vi "Check Events.vi"(8 "error in (no error)":errorcluster, 11 "PluginGUI in":refnum<class "PluginGUI.lvclass">) -> (0 "error out":errorcluster, 3 "PluginGUI out":refnum<class "PluginGUI.lvclass">)   [LabVIEW 2020, in "VolatusGUI.lvlib" / "PluginGUI.lvclass"]
uses:
  PluginGUI.lvclass
  C:/dev/lv20CE/relink/lv-volatus/Volatus/Module/Module.lvclass
  PluginGUI.lvclass/PluginGUI.ctl
  Volatus/Module/Module.lvclass/Module.ctl
  OnValueChangeHandler/OnValueChangeHandler.lvclass
  OnMouseDown/OnMouseDown.lvclass
  Volatus/Module/Module.lvclass
  Volatus/VolatusAPI/VolatusAPI.lvclass
  Volatus/Volatus.lvlib
  C:/dev/lv20CE/relink/lv-volatus/VolatusGUI/PluginGUI/PluginGUI.lvclass
  GUI Helper/GUI Helper.lvclass
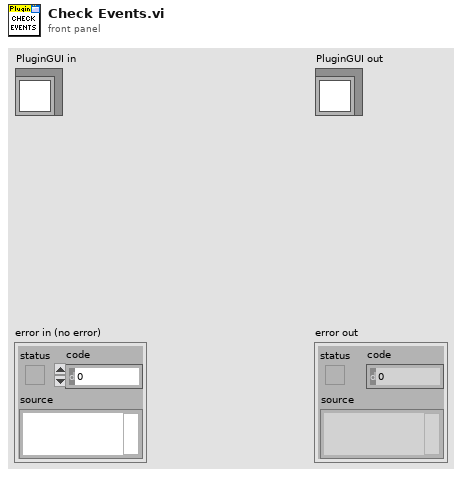
[diagram p1: front panel]
types:
  T1 = typedef "LVPoint32TypeDef.ctl" = cluster{"Horizontal":i32, "Vertical":i32}
  T2 = cluster{"Shift":bool, "Ctrl":bool, "Alt":bool, "Cmd":bool, "Opt":bool}
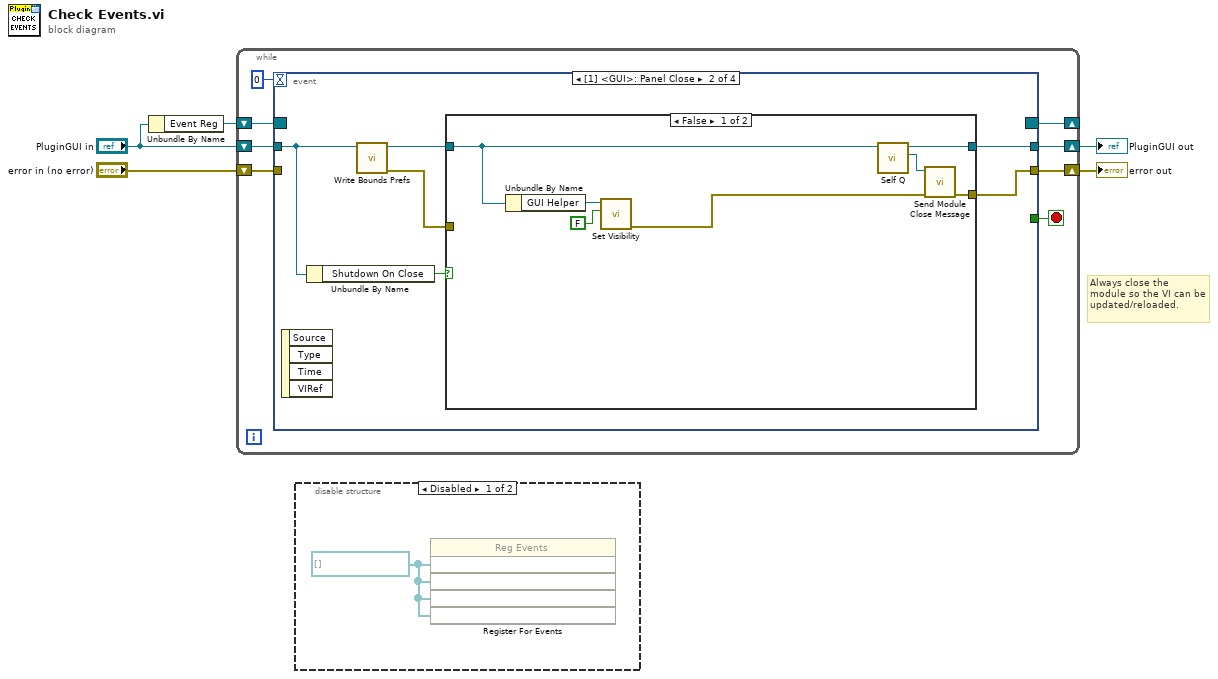
[diagram p0: block diagram]
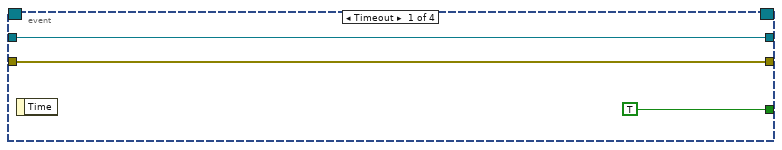
[diagram p3: hidden frame]
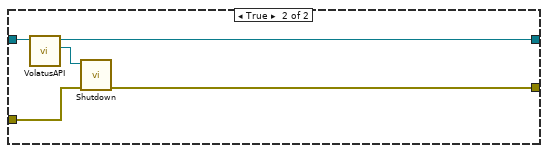
[diagram p4: hidden frame]
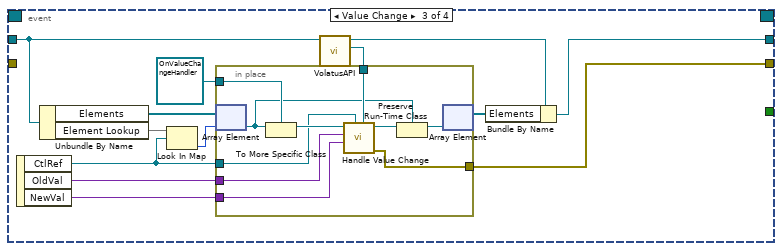
[diagram p5: hidden frame]
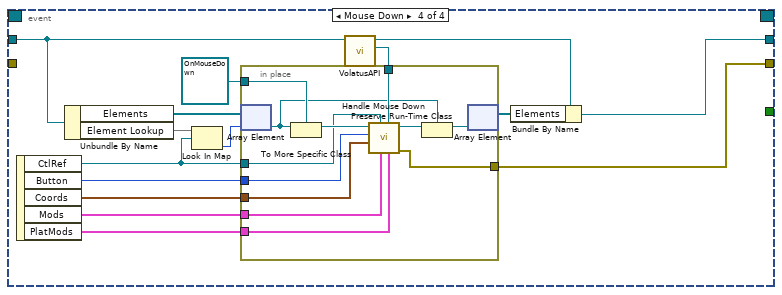
[diagram p6: hidden frame]
diagram:
  # "Always close the module so the VI can be updated/reloaded."
  n1 = Unbundle By Name("PluginGUI in") -> ("Event Reg"=w4:refnum<event-registration>)
  n2 = while {
    shift-right: [w8] -> w2
    shift-left: "PluginGUI in" -> [w11]
    shift-right: [w12] -> _
    shift-left: w4 -> [w13]
    shift-right: [w7] -> w1
    shift-left: "error in (no error)" -> [w10]
    stop <- w6 stop-if-true
    n3 = event shown="[1] <GUI>: Panel Close" {
      selector: w13 -> [_ _ _ _]
      dyn-events: [_ _ _ _] -> w12
      timeout: 0 -> [_ _ _ _]
      tunnel: w11 -> [w16 w21 w42 w58]
      tunnel: w10 -> [w15 _ _ _]
      tunnel: [w16 w20 w36 w64] -> w8
      tunnel: [w15 w19 w37 w65] -> w7
      tunnel: [TRUE _ _ _] -> w6
      event Timeout {
        n4 = event-data() -> ()  [unwired: 1 in, 1 out]
      }
      event Panel Close {
        n5 = event-data() -> ()  [unwired: 1 in, 4 out]
        n6 = Unbundle By Name(w21) -> ("Shutdown On Close"=w22:bool)
        n7 = call "Write Bounds Prefs.vi"("PluginGUI in"=w21) -> ("error out"=w17:errorcluster, "PluginGUI out"=w18:refnum<class "PluginGUI.lvclass">)  [unwired: 9 in]
        n8 = case shown="False" w22 {
          tunnel: w18 -> [w26 w34]
          tunnel: [w29 w32] -> w20
          tunnel: [w27 w31] -> w19
          tunnel: w17 -> [_ w30]
          frame False {
            n9 = Unbundle By Name(w26) -> ("GUI Helper"=w25:refnum<class "MessageQ.lvclass">)
            n10 = call "Set Visibility.vi"("Visible"=FALSE, "GUI Helper in"=w25) -> ("error out"=w23:errorcluster)  [unwired: 8 in, 1 out]
            n11 = call "Self Q.vi"("Module in"=w26) -> ("Self Q"=w28:refnum<class "MessageQ.lvclass">, "Module in"=w29:refnum<class "PluginGUI.lvclass">)  [unwired: 9 in]
            n12 = call "Send Module Close Message.vi"("error in (no error)"=w23, "MessageQ"=w28) -> ("error out"=w27:errorcluster)  [unwired: 9 in]
          }
          frame True {
            n13 = call "VolatusAPI.vi"("Module in"=w34) -> ("VolatusAPI"=w33:refnum<class "VolatusAPI.lvclass">, "Module in"=w32:refnum<class "PluginGUI.lvclass">)  [unwired: 9 in]
            n14 = call "Shutdown.vi"("error in (no error)"=w30, "VolatusAPI in"=w33) -> ("error out"=w31:errorcluster)  [unwired: 8 in, 1 out]
          }
        }
      }
      event Value Change {
        n15 = event-data() -> ("CtlRef"=w43:refnum<vi>, "OldVal"=w39:variant, "NewVal"=w38:variant)  [unwired: 1 in]
        n16 = Unbundle By Name(w42) -> ("Elements"=w46:refnum<class "GUI Element.lvclass">[], "Element Lookup"=w47:map{refnum<vi>, i32})
        n17 = Look In Map(map=w47, key=w43) -> (value=w45:i32)  [unwired: 1 in, 1 out]
        n18 = call "VolatusAPI.vi"("Module in"=w42) -> ("VolatusAPI"=w41:refnum<class "VolatusAPI.lvclass">, "Module in"=w40:refnum<class "PluginGUI.lvclass">)  [unwired: 9 in]
        n19 = in-place {
          in-place-border: refnum<class "OnValueChangeHandler.lvclass"> refnum ("OnValueChangeHandler in") -> [w56]
          in-place-border: w43 -> [w55]
          in-place-border: w41 -> [w54]
          in-place-border: w39 -> [w53]
          in-place-border: w38 -> [w52]
          in-place-border: [w48] -> w37
          n20 = in-place-array #1(w46, w45) -> (w49:refnum<class "GUI Element.lvclass">)
          n21 = To More Specific Class(target class=w56, reference=w49) -> (specific class reference=w57:refnum<class "OnValueChangeHandler.lvclass">)  [unwired: 1 in, 1 out]
          n22 = call-dynamic "Handle Value Change.vi"("VolatusAPI"=w54, "CtlRef"=w55, "NewVal"=w52, "OldVal"=w53, "OnValueChangeHandler in"=w57) -> ("error out"=w48:errorcluster, "OnValueChangeHandler out"=w51:refnum<class "OnValueChangeHandler.lvclass">)  [unwired: 5 in]
          n23 = Preserve Run-Time Class(object in=w51, 2:w49) -> (object out=w50:refnum<class "GUI Element.lvclass">)  [unwired: 1 in, 1 out]
          n24 = in-place-array #1(w50) -> (w35:refnum<class "GUI Element.lvclass">[])  [unwired: 1 out]
        }
        n25 = Bundle By Name(cluster=w40, "Elements"=w35) -> (w36:refnum<class "PluginGUI.lvclass">)
      }
      event Mouse Down {
        n26 = event-data() -> ("CtlRef"=w63:refnum<vi>, "Button"=w62:u16, "Coords"=w61:T1, "Mods"=w60:cluster{"Double Click":bool, "Menu Key":bool}, "PlatMods"=w59:T2)  [unwired: 1 in]
        n27 = Unbundle By Name(w58) -> ("Elements"=w71:refnum<class "GUI Element.lvclass">[], "Element Lookup"=w72:map{refnum<vi>, i32})
        n28 = Look In Map(map=w72, key=w63) -> (value=w70:i32)  [unwired: 1 in, 1 out]
        n29 = call "VolatusAPI.vi"("Module in"=w58) -> ("VolatusAPI"=w68:refnum<class "VolatusAPI.lvclass">, "Module in"=w67:refnum<class "PluginGUI.lvclass">)  [unwired: 9 in]
        n30 = in-place {
          in-place-border: refnum<class "OnMouseDown.lvclass"> refnum ("OnValueChangeHandler in") -> [w83]
          in-place-border: w63 -> [w82]
          in-place-border: w68 -> [w81]
          in-place-border: [w77] -> w65
          in-place-border: w62 -> [w76]
          in-place-border: w61 -> [w75]
          in-place-border: w60 -> [w74]
          in-place-border: w59 -> [w73]
          n31 = in-place-array #2(w71, w70) -> (w78:refnum<class "GUI Element.lvclass">)
          n32 = To More Specific Class(target class=w83, reference=w78) -> (specific class reference=w84:refnum<class "OnMouseDown.lvclass">)  [unwired: 1 in, 1 out]
          n33 = call-dynamic "Handle Mouse Down.vi"("PlatMods"=w73, "VolatusAPI"=w81, "Mods"=w74, "CtlRef"=w82, "Coords"=w75, "Button"=w76, "OnMouseDown in"=w84) -> ("error out"=w77:errorcluster, "OnMouseDown out"=w80:refnum<class "OnMouseDown.lvclass">)  [unwired: 3 in]
          n34 = Preserve Run-Time Class(object in=w80, 2:w78) -> (object out=w79:refnum<class "GUI Element.lvclass">)  [unwired: 1 in, 1 out]
          n35 = in-place-array #2(w79) -> (w66:refnum<class "GUI Element.lvclass">[])  [unwired: 1 out]
        }
        n36 = Bundle By Name(cluster=w67, "Elements"=w66) -> (w64:refnum<class "PluginGUI.lvclass">)
      }
    }
  }
  "error out" <- w1
  "PluginGUI out" <- w2
  n37 = disable-structure shown="Disabled" {
    frame Disabled {
      w85 = refnum<vi>[] []
      n38 = register-events(w85, w85, w85, w85) -> ()  [unwired: 2 in, 2 out]
    }
    frame Enabled {
    }
  }
